vi "publish.vi"(8 "error in":errorcluster, 9 "Python env version":string="3.12", 10 "Path to service.py":path, 11 "Python env directory":path) -> (0 "error out":errorcluster)   [LabVIEW 2023]
uses:
  <vilib>/Python/Open Venv Python Session.vi
panel:
  out "value":i32
  in  "Process Stop Button":bool
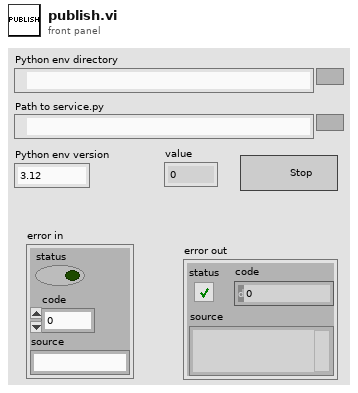
[diagram p1: front panel]
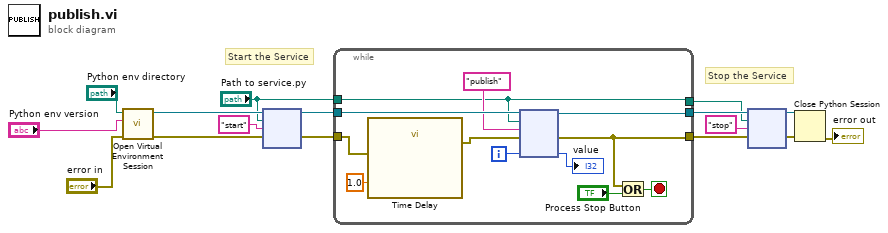
[diagram p0: block diagram]
diagram:
  # "Stop the Service"
  # "Start the Service"
  n1 = call-poly <vilib>:"Open Virtual Environment Session.vi"("error in (no error)"="error in", "Python version"="Python env version", "Env path"="Python env directory") -> ("error out"=w13:errorcluster, "session out"=w14:refnum<k35>)  [unwired: 7 in]
  n2 = node(w14, "Path to service.py", "start" ("function name"), w13) -> (w10:refnum<k35>, w11:errorcluster)  [unwired: 2 in, 2 out]
  n3 = while {
    tunnel: w11 -> [w26]
    tunnel: w10 -> [w25]
    tunnel: [w23] -> w9
    tunnel: [w17] -> w8
    tunnel: "Path to service.py" -> [w19]
    tunnel: [w19] -> w5
    i -> [w24]
    stop <- w28 stop-if-true
    n4 = call "Time Delay"("error in (no error)"=w26, "Delay Time (s)"=1.0) -> ("error out"=w18:errorcluster)  [unwired: 9 in]
    n5 = node(w25, w19, "publish" ("function name"), w18, w24) -> (w23:refnum<k35>, w17:errorcluster, →"value":i32)  [unwired: 2 in, 2 out]
    n6 = Or(x=w17, y="Process Stop Button") -> (x .or. y?=w28:bool)
  }
  n7 = node(w9, w5, "stop" ("function name"), w8) -> (w4:refnum<k35>, w1:errorcluster)  [unwired: 2 in, 2 out]
  n8 = Close Python Session(session in=w4, error in=w1) -> (11:→"error out":errorcluster)
